vi "Task Init.vi"(8 "error in (no error)":errorcluster, 11 "SimTask in":refnum<class "SimTask.lvclass">) -> (0 "error out":errorcluster, 3 "SimTask out":refnum<class "SimTask.lvclass">)   [LabVIEW 2020, in "VolatusDemo.lvlib" / "SimTask.lvclass"]
uses:
  SimTask.lvclass
  Volatus/Task/Task.lvclass/Task.ctl
  SimTask.lvclass/SimTask.ctl
  Volatus/TelemetryAPI/Create Group.vi
  Volatus/Task/Task.lvclass
  lv-vecto/Vecto/Group/Group.lvclass
  C:/dev/lv20CE/relink/lv-volatus/Volatus/Task/Task.lvclass
  C:/Program Files (x86)/National Instruments/LabVIEW 2020/vi.lib/ActorFramework/Actor/Actor.lvclass
  C:/dev/lv20CE/relink/lv-volatus/Volatus/APIRegistrationHandler/APIRegistrationHandler.lvclass
  C:/dev/lv20CE/relink/lv-volatus/Volatus/TaskStateHandler/TaskStateHandler.lvclass
  C:/dev/lv20CE/relink/lv-volatus/Volatus/VectoMessageHandler/VectoMessageHandler.lvclass
  C:/dev/lv20CE/relink/lv-volatus/VolatusDemo/SimTask/SimTask.lvclass
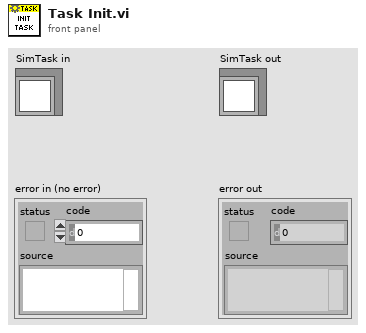
[diagram p1: front panel]
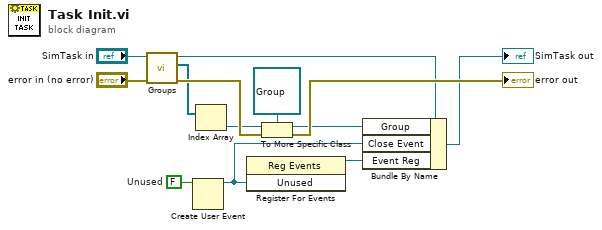
[diagram p0: block diagram]
diagram:
  w11 = FALSE  # Unused
  n1 = call "Groups.vi"("error in (no error)"="error in (no error)", "Task in"="SimTask in") -> ("error out"=w13:errorcluster, "Groups"=w6:refnum<class "GroupAbstract.lvclass">[], "Task out"=w4:refnum<class "SimTask.lvclass">)  [unwired: 7 in]
  n2 = Create User Event(user event datatype=w11) -> (user event=w9:refnum<user-event>)  [unwired: 1 in, 1 out]
  n3 = Index Array(array=w6) -> (element=w5:refnum<class "GroupAbstract.lvclass">)  [unwired: 1 in]
  n4 = register-events(w9) -> (reference out=w10:refnum<event-registration>)  [unwired: 2 in, 1 out]
  n5 = To More Specific Class(target class=refnum<class "Group.lvclass"> refnum ("Vecto.lvlib:Group.lvclass"), reference=w5, error in=w13) -> (specific class reference=w3:refnum<class "Group.lvclass">, error out=→"error out":errorcluster)
  n6 = Bundle By Name(cluster=w4, "Group"=w3, "Close Event"=w9, "Event Reg"=w10) -> (→"SimTask out":refnum<class "SimTask.lvclass">)
